vi "VIH Constant - Default Build Root Folder.vi"() -> (3 "Default Build Root Folder":path)   [LabVIEW 2014]
doc: "::: VI Helpeks :::\nCopyright (c) 2000-2026 Konstantin Shifershteyn. All rights reserved."
panel:
  # "VI Helpeks\nCopyright (c) 2012-2026 Konstantin Shifershteyn"
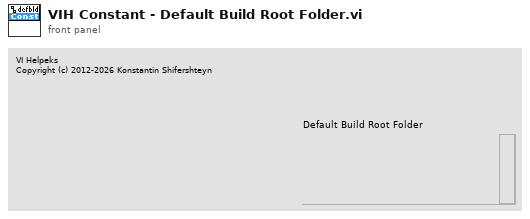
[diagram p1: front panel]
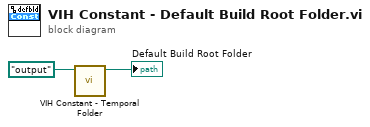
[diagram p0: block diagram]
diagram:
  n1 = call "VIH Constant - Temporal Folder.vi"("append path"=path "output") -> ("Temporal folder"=→"Default Build Root Folder":path)  [unwired: 10 in]
